vi "SimuladorTemperaturaCSV.vi"() -> ()   [LabVIEW 2025]
panel:
  out "Contador":i32=8
  in  "Ubicación":path=path "C:/Users/oscar/OneDrive - Instituto Politecnico Nacional/Documents/I+D - Libros/Proyectos/DAQs/Simulacion_1_CSV_LabVIEW/Datos.csv"
  in  "stop":bool
  out "Temperatura":dbl=24.69722162669874
  out "Temperatura Chart":dbl(graph)=24.69722162669874
  out "Termómetro":dbl(slide)=24.69722162669874 scale=0.0..100.0
  in  "Periodo":u32=1000
  in  "Ruido":dbl=0.5
  in  "Knob":dbl(knob)=24.65591787788892 scale=0.0..60.0
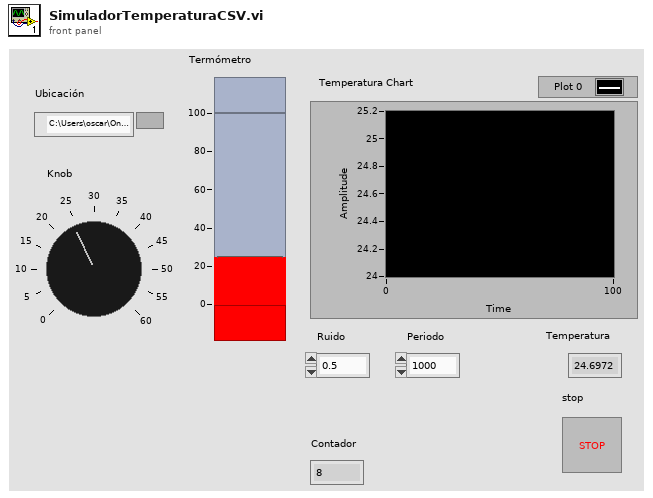
[diagram p1: front panel]
types:
  T1 = enum16{"open", "replace", "create", "open or create", "replace or create", "replace or create with confirmation"}
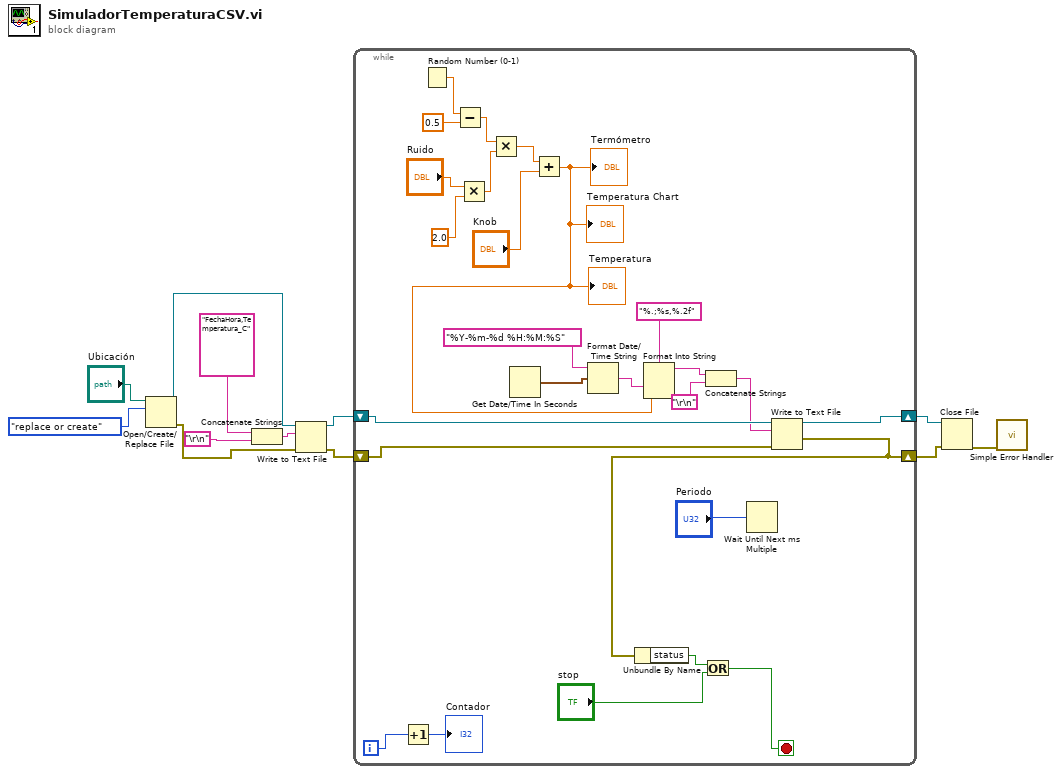
[diagram p0: block diagram]
diagram:
  n1 = Open/Create/Replace File(file path (use dialog)="Ubicación", operation (0:open)=T1."replace or create") -> (refnum out=w7:refnum<file>, error out=w6:errorcluster)  [unwired: 4 in, 1 out]
  n2 = Concatenate Strings("FechaHora,Temperatura_C", "\r\n") -> (w8:string)
  n3 = Write to Text File(file (use dialog)=w7, text=w8, error in=w6) -> (refnum out=w5:refnum<file>, error out=w4:errorcluster)  [unwired: 1 in, 1 out]
  n4 = while {
    shift-right: [w26] -> w3
    shift-left: w5 -> [w28]
    shift-right: [w22] -> w2
    shift-left: w4 -> [w27]
    i -> [w25]
    stop <- w19 stop-if-true
    n5 = Increment(x=w25) -> (x+1=→"Contador":i32)
    n6 = Random Number (0-1)() -> (number: 0 to 1=w38:dbl)
    n7 = Subtract(x=w38, y=0.5) -> (x-y=w36:dbl)
    n8 = Multiply(x="Ruido", y=2.0) -> (x*y=w33:dbl)
    n9 = Multiply(x=w36, y=w33) -> (x*y=w32:dbl)
    n10 = Get Date/Time In Seconds() -> (seconds since 1Jan1904=w29:timestamp)
    n11 = Add(x=w32, y="Knob") -> (x+y=w16:dbl)
    "Termómetro" <- w16
    "Temperatura Chart" <- w16
    "Temperatura" <- w16
    n12 = Format Date/Time String(time format string (%c)="%Y-%m-%d %H:%M:%S", seconds (now)=w29) -> (date/time string=w17:string)  [unwired: 1 in]
    n13 = Format Into String(format string="%.;%s,%.2f", w17, w16) -> (resulting string=w15:string)  [unwired: 2 in, 1 out]
    n14 = Concatenate Strings(w15, "\r\n") -> (w13:string)
    n15 = Wait Until Next ms Multiple(millisecond multiple="Periodo") -> ()  [unwired: 1 out]
    n16 = Write to Text File(file (use dialog)=w28, text=w13, error in=w27) -> (refnum out=w26:refnum<file>, error out=w22:errorcluster)  [unwired: 1 in, 1 out]
    n17 = Unbundle By Name(w22) -> ("status"=w21:bool)
    n18 = Or(x=w21, y="stop") -> (x .or. y?=w19:bool)
  }
  n19 = Close File(refnum=w3, error in=w2) -> (error out=w1:errorcluster)  [unwired: 1 out]
  n20 = call <vilib>:"Simple Error Handler.vi"("error in (no error)"=w1) -> ()  [unwired: 4 in, 5 out]
